vi "Update CAN Status.vi"(8 "error in (no error)":errorcluster, 11 "CAN RW CANsub in":refnum<class "CAN RW CANsub.lvclass">) -> (0 "error out":errorcluster, 3 "CAN RW CANsub out":refnum<class "CAN RW CANsub.lvclass">)   [LabVIEW 2021, in "CAN RW CANsub.lvclass"]
doc: "Reads the CAN status of the channel from the device (REST) and stores it for the CAN Status accessor. Makes the REST call one time in each second at most; at other times the stored status stays. A failed REST call gives no error: the stored status stays and the next call comes after 5 s. After 60 s with no status: error 5303. If the device reports the channel as stopped: error 5304. The REST call has a time limit of 500 ms. Loop-safe when no call is due."
uses:
  CAN RW CANsub.lvclass
  CAN RW CANsub.lvclass/CAN RW CANsub.ctl
  CANsub/c_client/api/CANsub_Channel/CANsub_Channel.lvclass
  <vilib>/CIF Foundation/CIF CAN RW Core/CAN_RW_CORE.lvclass
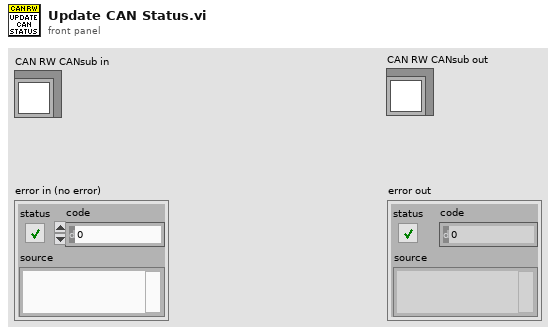
[diagram p1: front panel]
types:
  T1 = typedef "CANsub_Common.lvlib/CANsub_Device_Status.ctl" = cluster{"state":string, "frame_count":u32, "frame_rate":dbl, "bus_load":dbl, "rx_error_count":u32, "tx_error_count":u32, "bus_error_count":u32}
  T2 = typedef "CAN_RW_CORE.lvclass/CAN Status.ctl" = cluster{"Comm State":T3, "Last Error":T4, "RX Error Counter":u8, "TX Error Counter":u8}
  T3 = typedef "CAN_RW_CORE.lvclass/Communication State.ctl" = enum16{"Error Active", "Error Passive", "Bus Off"}
  T4 = typedef "CAN_RW_CORE.lvclass/Last Error.ctl" = enum16{"None", "Stuff", "Form", "Ack", "Bit1", "Bit0", "CRC", "Unknown"}
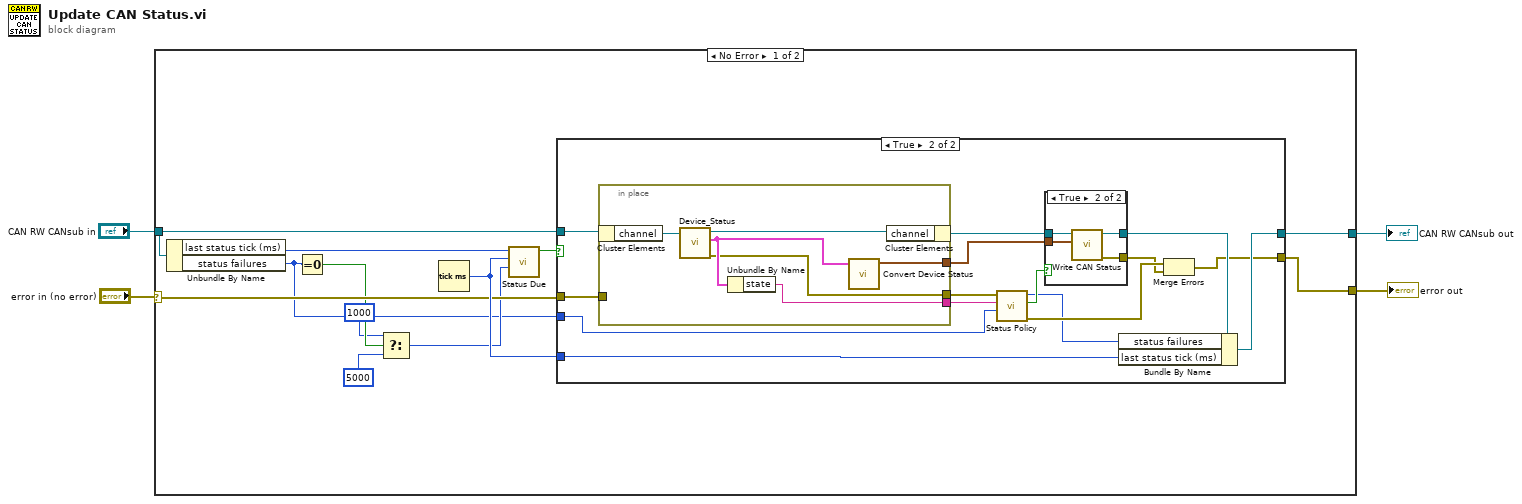
[diagram p0: block diagram]
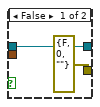
[diagram p3: hidden frame]
diagram:
  n1 = case shown="No Error" "error in (no error)" {
    selector: "error in (no error)" -> [w10 w46]
    tunnel: [w16 w47] -> w4
    tunnel: [w15 w46] -> w3
    tunnel: "CAN RW CANsub in" -> [w13 w47]
    frame No Error {
      n2 = Unbundle By Name(w13) -> ("last status tick (ms)"=w12:u32, "status failures"=w5:u32)
      n3 = Equal To 0?(x=w5) -> (x = 0?=w9:bool)
      n4 = Select(t=u32 1000, s=w9, f=u32 5000) -> (s? t:f=w6:u32)
      n5 = Tick Count (ms)() -> (millisecond timer value=w11:u32)
      n6 = call "Status Due.vi"("interval (ms)"=w6, "now (ms)"=w11, "last tick (ms)"=w12) -> ("due"=w14:bool)  [unwired: 8 in]
      n7 = case shown="True" w14 {
        tunnel: w13 -> [w18 w33]
        tunnel: w10 -> [w17 w32]
        tunnel: [w18 w28] -> w16
        tunnel: [w17 w19] -> w15
        tunnel: w11 -> [_ w27]
        tunnel: w5 -> [_ w26]
        frame False {
        }
        frame True {
          n8 = in-place {
            in-place-border: w32 -> [_]
            in-place-border: [w43] -> w30
            in-place-border: [w41] -> w24
            in-place-border: [w40] -> w25
            n9 = in-place-cluster #1(w33) -> ("channel"=w45:refnum<class "CANsub_Channel.lvclass">)
            n10 = call-dynamic "Device_Status.vi"("CANsub_Channel in"=w45) -> ("error out"=w41:errorcluster, "device status"=w42:T1, "CANsub_Channel out"=w44:refnum<class "CANsub_Channel.lvclass">)  [unwired: 8 in]
            n11 = Unbundle By Name(w42) -> ("state"=w40:string)
            n12 = call "Convert Device Status.vi"("device status"=w42) -> ("CAN Status"=w43:T2)  [unwired: 10 in]
            n13 = in-place-cluster #1("channel"=w44) -> (w31:refnum<class "CAN RW CANsub.lvclass">)
          }
          n14 = call "Status Policy.vi"("failures in"=w26, "state"=w25, "call error"=w24) -> ("error out"=w22:errorcluster, "update status"=w23:bool, "failures out"=w20:u32)  [unwired: 6 in]
          n15 = case shown="True" w23 {
            tunnel: w31 -> [w35 w39]
            tunnel: w30 -> [_ w38]
            tunnel: [errorcluster {"status"=FALSE, "code"=0, "source"=""} ("error out") w37] -> w21
            tunnel: [w35 w36] -> w29
            frame False {
            }
            frame True {
              n16 = call <vilib>:"Write CAN Status.vi"("CAN Status"=w38, "CAN_RW_CORE in"=w39) -> ("error out"=w37:errorcluster, "CAN_RW_CORE out"=w36:refnum<class "CAN RW CANsub.lvclass">)  [unwired: 8 in]
            }
          }
          n17 = Bundle By Name(cluster=w29, "status failures"=w20, "last status tick (ms)"=w27) -> (w28:refnum<class "CAN RW CANsub.lvclass">)
          n18 = Merge Errors(w22, w21) -> (w19:errorcluster)
        }
      }
    }
    frame Error {
    }
  }
  "CAN RW CANsub out" <- w4
  "error out" <- w3
